vi "GetAllMethodsTypesForClass.vi"(0 "ClassWriterNative":refnum<class "ClassWriterNative.lvclass">, 5 "ClassItemRefIn":refnum<vi>, 11 "error in":errorcluster) -> (2 "MethodTemplatePathOut":path, 3 "DesignPattern":T5[](array[typedef]), 4 "NormalMethods":T2[](array[typedef]), 6 "OverrideMethods":T2[](array[typedef]), 8 "PropertyMethods":T2[](array[typedef]), 10 "ConnectorPaneHeight":i32[](array[numeric]), 13 "TemplateSettings":T1, 14 "PropertyNodeMethods":T2[](array[typedef]), 15 "error out":errorcluster)   [LabVIEW 2020, in "ClassWriterNative.lvclass"]
uses:
  <resource>/Framework/Providers/Open_GDS/ClassProviders/Provider_LvNativeClass/ClassWriterNative_class/ClassWriterNative.lvclass
  <resource>/Framework/Providers/Open_GDS/ClassProviders/Provider_LvNativeClass/ClassWriterNative_class/MethodInfo.ctl
  <resource>/Framework/Providers/Open_GDS/ClassProviders/Provider_LvNativeClass/ClassWriterNative_class/MethodType.ctl
  <resource>/Framework/Providers/Open_GDS/ClassProviders/Provider_LvNativeClass/ClassWriterNative_class/MethodInfo_Option.ctl
  <resource>/Framework/Providers/Open_GDS/ClassProviders/Common/LvClass_class/GDSLvClass_PlugIn.ctl
  <resource>/Framework/Providers/Open_GDS/ClassProviders/Common/LvClass_class/GDSLvClass_PlugInTypes.ctl
  <resource>/Framework/Providers/Open_GDS/ClassProviders/Provider_BaseClassInterface/ClassWriter_class/TemplateSettings.ctl
  <resource>/Framework/Providers/Open_GDS/ClassProviders/Provider_BaseClassInterface/BaseProvider_SubVIs/BaseProvider_PlugInManagerActions.ctl
  <resource>/Framework/Providers/Open_GDS/ClassProviders/Provider_LvNativeClass/ClassWriterNative_class/ClassWriterNative.lvclass/ClassWriterNative.ctl
  <resource>/Framework/Providers/Open_GDS/ClassProviders/Provider_BaseClassInterface/ClassWriter_class/ClassWriter.lvclass
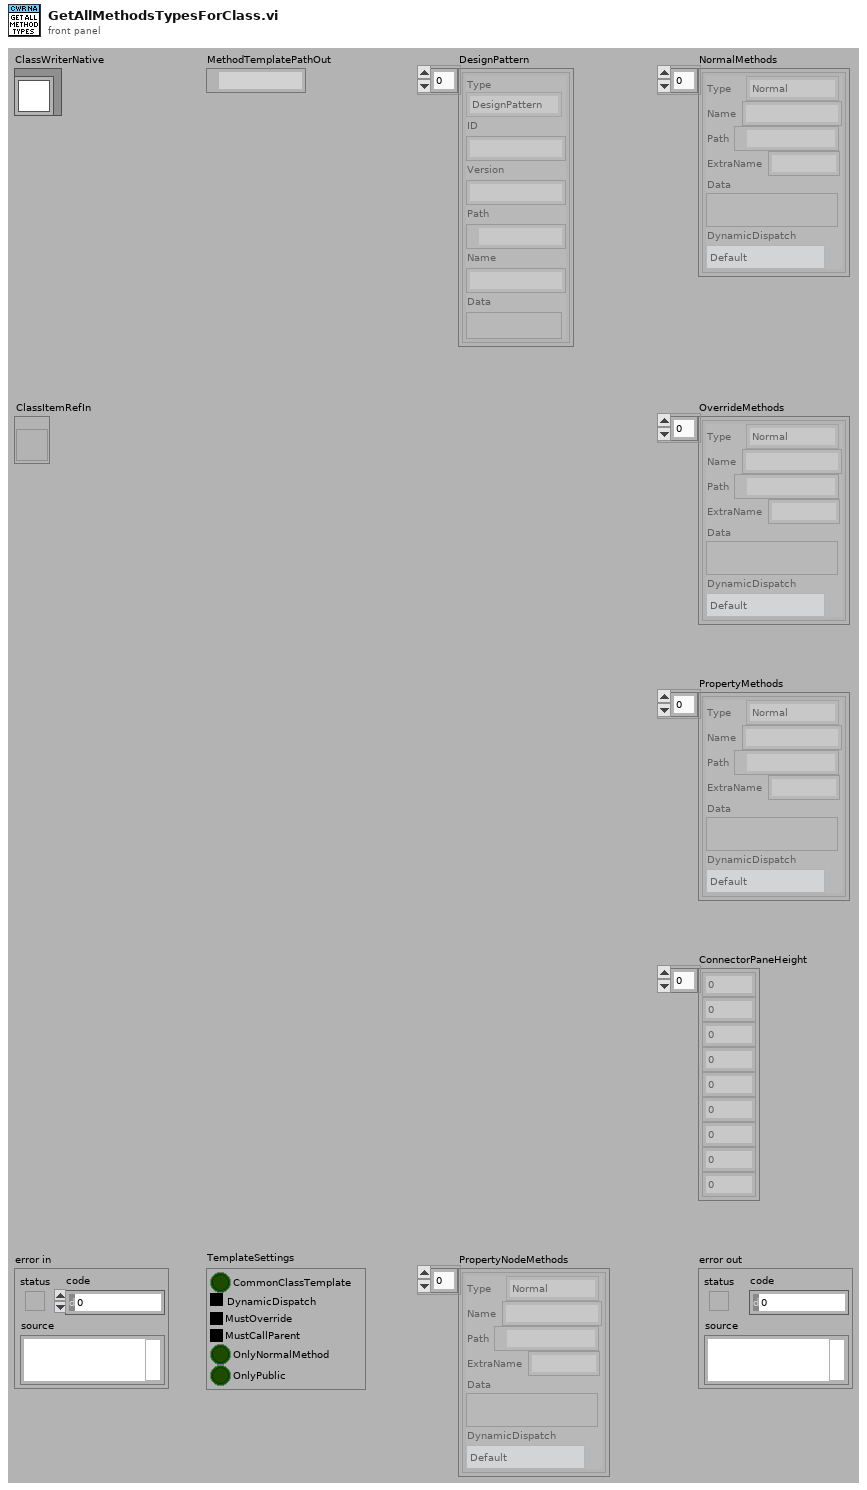
[diagram p1: front panel]
types:
  T1 = typedef "ClassWriter.lvclass/TemplateSettings.ctl" = cluster{"CommonClassTemplate":bool, "DynamicDispatch":enum8{"False", "True", "Mixed"}, "MustOverride":enum8{"False", "True", "Mixed"}, "MustCallParent":enum8{"False", "True", "Mixed"}, "OnlyNormalMethod":bool, "OnlyPublic":bool}
  T2 = typedef "ClassWriterNative.lvclass/MethodInfo.ctl" = cluster{"Type":T3, "Name":string, "Path":path, "ExtraName":string, "Data":variant, "DynamicDispatch":T4}
  T3 = typedef "ClassWriterNative.lvclass/MethodType.ctl" = enum16{"Normal", "MethodPlugIn", "DesignPattern", "AF-Method"}
  T4 = typedef "ClassWriterNative.lvclass/MethodInfo_Option.ctl" = enum16{"Default", "OnAtStart", "OffAtStart", "AlwaysOn", "AlwaysOff"}
  T5 = typedef "GDSLvClass_PlugIn.ctl" = cluster{"Type":T6, "ID":string, "Version":string, "Path":path, "Name":string, "Data":variant}
  T6 = typedef "GDSLvClass_PlugInTypes.ctl" = enum16{"DesignPattern", "MethodTypes"}
  T7 = typedef "GDSLvCLass_ClassSettingsType.ctl" = cluster{"ClassProviderName":string, "ClassTemplateUsed":string, "ClassTemplateVersion":string, "ClassDescription":string, "PlugIns":T5[], "ConnectorPanePattern":string}
  T8 = typedef "BaseProvider_PlugInManagerActions.ctl" = enum16{"GetPluginsMethods", "ExecutePlugIn"}
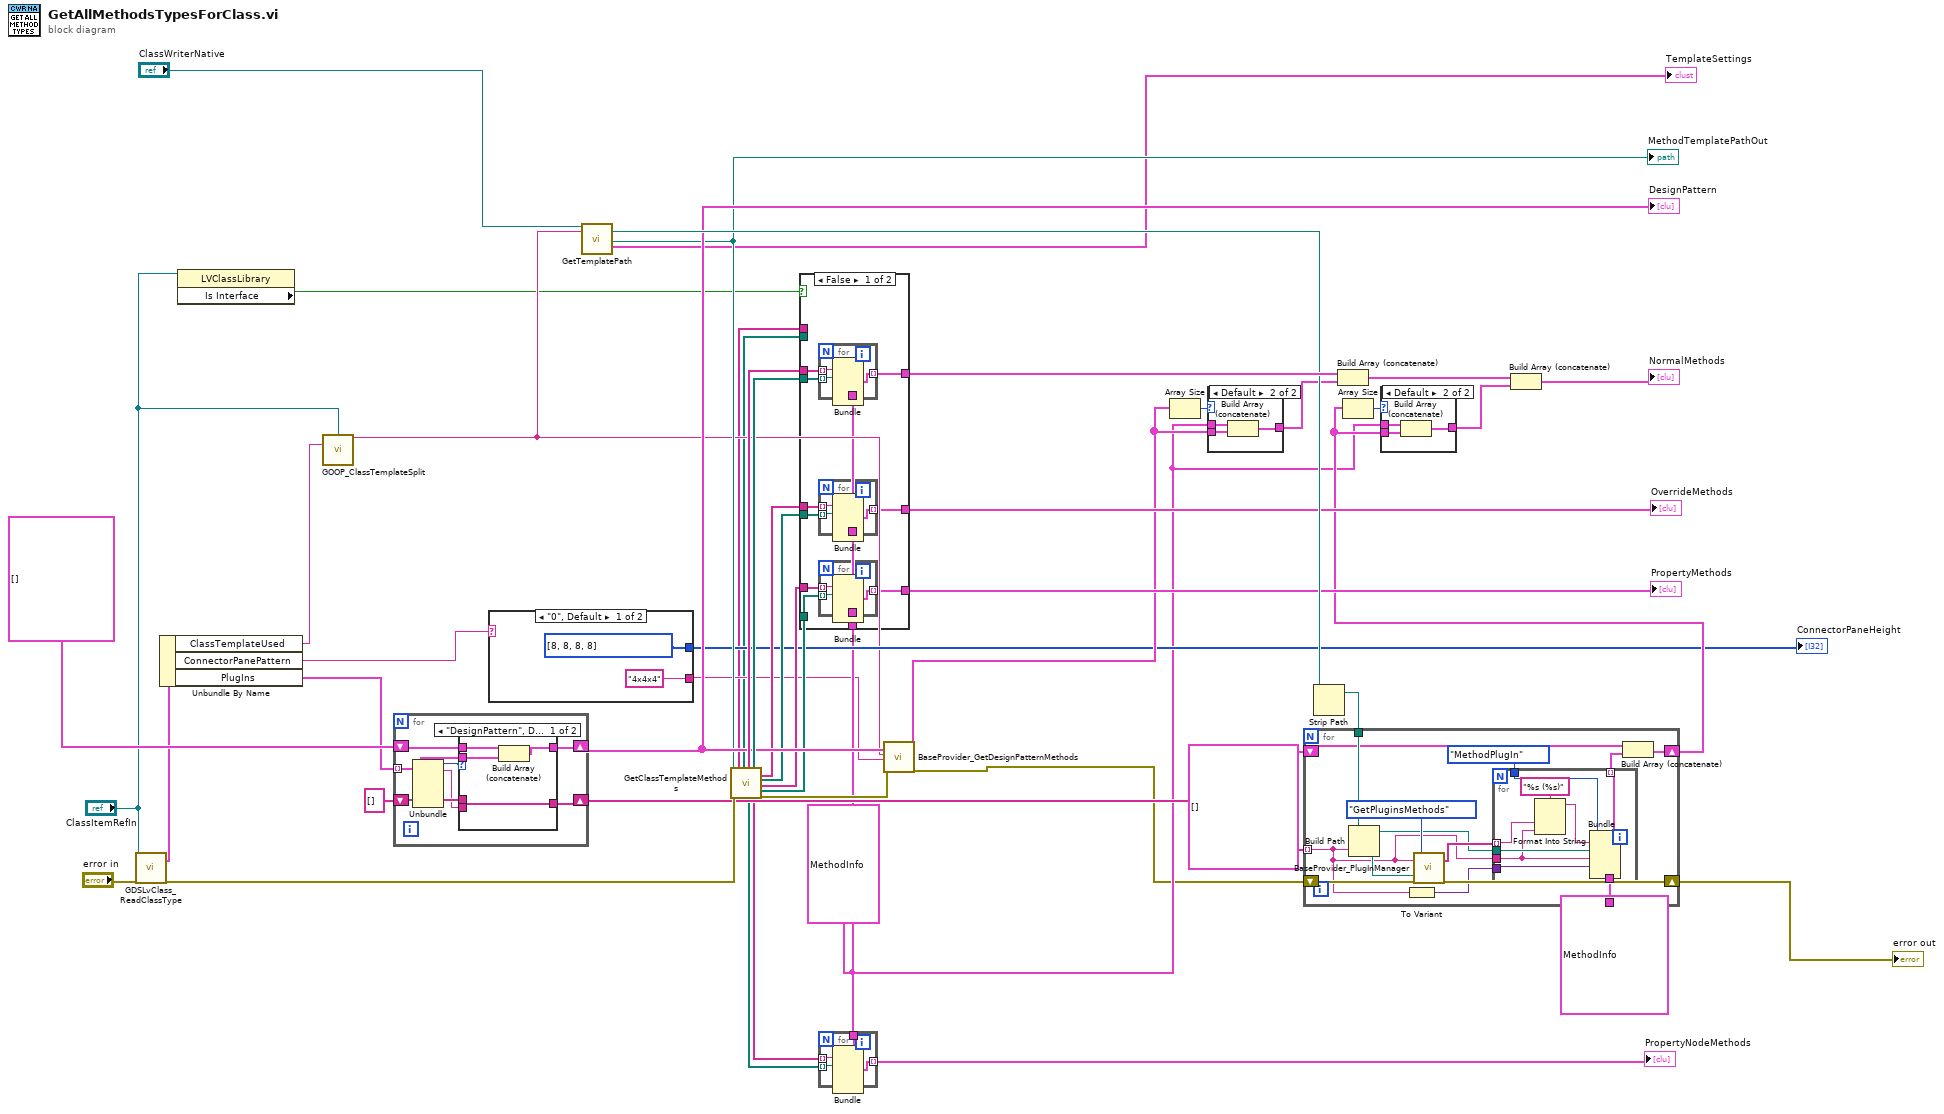
[diagram p0: block diagram]
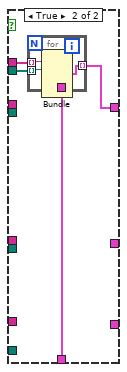
[diagram p2: hidden frame]
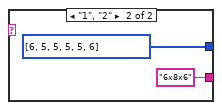
[diagram p3: hidden frame]
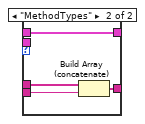
[diagram p6: hidden frame]
diagram:
  w12 = T2 {"Type"=enum."Normal", "Name"="", "Path"=path "", "ExtraName"="", "Data"=variant, "DynamicDispatch"=enum."Default"} ("Cluster")
  n1 = call <resource>:"GDSLvClass_ReadClassType.vi"("Class Refnum In"="ClassItemRefIn", "error in (no error)"="error in") -> ("ClassSettings"=w34:T7, "error out"=w47:errorcluster)  [unwired: 15 in, 1 out]
  n2 = Unbundle By Name(w34) -> ("ClassTemplateUsed"=w14:string, "ConnectorPanePattern"=w13:string, "PlugIns"=w36:T5[])
  n3 = property class="LVClassLibrary"(reference="ClassItemRefIn") -> ("Is Interface"=w3:bool)  [unwired: 1 in, 2 out]
  n4 = call <resource>:"GOOP_ClassTemplateSplit.vi"("ClassItemRefIn"="ClassItemRefIn", "FullClassTemplate"=w14) -> ("StandardTemplate"=w6:string)  [unwired: 12 in, 1 out]
  n5 = for {
    tunnel: w36 -> [w49] mode=indexing
    shift-right: [w53] -> w42
    shift-left: string[] [] -> [w54]
    shift-right: [w50] -> w38
    shift-left: T5[] [] -> [w51]
    n6 = Unbundle(w49) -> ("Type"=w55:T6, "ID"=w52:string)  [unwired: 4 out]
    n7 = case shown="\"DesignPattern\", Default" w55 {
      tunnel: w54 -> [w59 w63]
      tunnel: [w59 w62] -> w53
      tunnel: w52 -> [_ w61]
      tunnel: w51 -> [w58 w60]
      tunnel: [w57 w60] -> w50
      tunnel: w49 -> [w56 _]
      frame "DesignPattern", Default {
        n8 = Build Array (concatenate)(w58, w56) -> (w57:T5[])
      }
      frame "MethodTypes" {
        n9 = Build Array (concatenate)(w63, w61) -> (w62:string[])
      }
    }
  }
  "DesignPattern" <- w38
  n10 = case shown="\"0\", Default" w13 {
    tunnel: ["4x4x4" "6x8x6"] -> w7
    tunnel: [i32[] [8, 8, 8, 8] ("ConnectorPaneHeight") i32[] [6, 5, 5, 5, 5, 6] ("ConnectorPaneHeight")] -> w15
    frame "0", Default {
    }
    frame "1", "2" {
    }
  }
  "ConnectorPaneHeight" <- w15
  n11 = call-dynamic "GetTemplatePath.vi"("reference in"="ClassWriterNative", "ClassTemplateSubDirectory"=w6) -> ("FolderPathOut"=w40:path, "MethodTemplatePathOut"=w25:path, "TemplateSettings"=→"TemplateSettings":T1)  [unwired: 13 in, 2 out]
  "MethodTemplatePathOut" <- w25
  n12 = call <resource>:"GetClassTemplateMethods.vi"("MethodTemplatePath"=w25, "error in"=w47) -> ("InterfaceMethodNames"=w2:string[], "InterfaceMethodPaths"=w1:path[], "NormalMethodNames"=w43:string[], "PropertyNodeMethodPaths"=w10:path[], "NormalMethodPaths"=w44:path[], "PropertyNodeMethodNames"=w11:string[], "OverrideMethodNames"=w33:string[], "OverrideMethodPaths"=w32:path[], "PropertyMethodNames"=w30:string[], "PropertyMethodPaths"=w29:path[], "error out"=w48:errorcluster)  [unwired: 7 in]
  n13 = case shown="False" w3 {
    tunnel: [w77 w90] -> w45
    tunnel: w44 -> [w76 _]
    tunnel: w43 -> [w75 _]
    tunnel: w33 -> [w74 _]
    tunnel: w32 -> [w73 _]
    tunnel: [w72 _] -> w31
    tunnel: w30 -> [w71 _]
    tunnel: w29 -> [w70 _]
    tunnel: [w69 _] -> w28
    tunnel: w12 -> [w68 w93]
    tunnel: w2 -> [_ w92]
    tunnel: w1 -> [_ w91]
    frame False {
      n14 = for {
        tunnel: w75 -> [w88] mode=indexing
        tunnel: w76 -> [w87] mode=indexing
        tunnel: w68 -> [w89]
        tunnel: [w86] -> w77 mode=indexing
        n15 = Bundle(cluster=w89, "Name"=w88, "Path"=w87) -> (w86:T2)  [unwired: 4 in]
      }
      n16 = for {
        tunnel: w74 -> [w84] mode=indexing
        tunnel: w73 -> [w83] mode=indexing
        tunnel: w68 -> [w85]
        tunnel: [w82] -> w72 mode=indexing
        n17 = Bundle(cluster=w85, "Name"=w84, "Path"=w83) -> (w82:T2)  [unwired: 4 in]
      }
      n18 = for {
        tunnel: w71 -> [w80] mode=indexing
        tunnel: w70 -> [w79] mode=indexing
        tunnel: w68 -> [w81]
        tunnel: [w78] -> w69 mode=indexing
        n19 = Bundle(cluster=w81, "Name"=w80, "Path"=w79) -> (w78:T2)  [unwired: 4 in]
      }
    }
    frame True {
      n20 = for {
        tunnel: w92 -> [w96] mode=indexing
        tunnel: w91 -> [w95] mode=indexing
        tunnel: w93 -> [w97]
        tunnel: [w94] -> w90 mode=indexing
        n21 = Bundle(cluster=w97, "Name"=w96, "Path"=w95) -> (w94:T2)  [unwired: 4 in]
      }
    }
  }
  "OverrideMethods" <- w31
  "PropertyMethods" <- w28
  n22 = for {
    tunnel: w11 -> [w100] mode=indexing
    tunnel: w10 -> [w99] mode=indexing
    tunnel: w12 -> [w101]
    tunnel: [w98] -> w9 mode=indexing
    n23 = Bundle(cluster=w101, "Name"=w100, "Path"=w99) -> (w98:T2)  [unwired: 4 in]
  }
  "PropertyNodeMethods" <- w9
  n24 = call <resource>:"BaseProvider_GetDesignPatternMethods.vi"("DesignPattern"=w38, "ClassTemplateName"=w6, "ConnectorPaneSettings"=w7, "error in"=w48) -> ("NormalMethods"=w17:T2[], "error out"=w8:errorcluster)  [unwired: 14 in]
  n25 = Array Size(array=w17) -> (size(s)=w27:i32)
  n26 = case shown="Default" w27 {
    tunnel: w17 -> [w102 w105]
    tunnel: [w102 w104] -> w26
    tunnel: w12 -> [_ w103]
    frame 0 {
    }
    frame Default {
      n27 = Build Array (concatenate)(w103, w105) -> (w104:T2[])
    }
  }
  n28 = Strip Path(path=w40) -> (stripped path=w41:path)  [unwired: 1 out]
  n29 = for {
    shift-right: [w117] -> w46
    shift-left: w8 -> [w116]
    tunnel: w42 -> [w106] mode=indexing
    tunnel: w41 -> [w115]
    shift-right: [w113] -> w18
    shift-left: T2[] [] -> [w114]
    tunnel: T2 {"Type"=enum."MethodPlugIn", "Name"="", "Path"=path "", "ExtraName"="", "Data"=variant, "DynamicDispatch"=enum."Default"} ("Cluster") -> [w112]
    n30 = Build Path(base path=w115, name or relative path=w106) -> (appended path=w108:path)
    n31 = To Variant(anything=w106) -> (Variant=w107:variant)
    n32 = call <resource>:"BaseProvider_PlugInManager.vi"("PlugInName"=w106, "PlugInPath"=w108, "error in (no error)"=w116, "Action"=BaseProvider_PlugInManagerActions."GetPluginsMethods") -> ("MethodsTypes"=w111:string[], "error out"=w117:errorcluster)  [unwired: 14 in]
    n33 = for {
      tunnel: w111 -> [w121] mode=indexing
      tunnel: w112 -> [w127]
      tunnel: [w126] -> w110 mode=indexing
      tunnel: w107 -> [w123]
      tunnel: MethodType."MethodPlugIn" ("Type") -> [w125]
      tunnel: w108 -> [w124]
      tunnel: w106 -> [w120]
      n34 = Format Into String(format string="%s (%s)", w121, w120) -> (resulting string=w119:string)  [unwired: 2 in, 1 out]
      n35 = Bundle(cluster=w127, "Type"=w125, "Name"=w119, "Path"=w124, "ExtraName"=w120, "Data"=w123) -> (w126:T2)  [unwired: 1 in]
    }
    n36 = Build Array (concatenate)(w114, w110) -> (w113:T2[])
  }
  "error out" <- w46
  n37 = Build Array (concatenate)(w45, w26) -> (w23:T2[])
  n38 = Array Size(array=w18) -> (size(s)=w24:i32)
  n39 = case shown="Default" w24 {
    tunnel: [w128 w131] -> w19
    tunnel: w18 -> [w128 w130]
    tunnel: w12 -> [_ w129]
    frame 0 {
    }
    frame Default {
      n40 = Build Array (concatenate)(w129, w130) -> (w131:T2[])
    }
  }
  n41 = Build Array (concatenate)(w23, w19) -> (→"NormalMethods":T2[])
